vi "TS Acq Start.vi"(8 "error in":errorcluster, 11 "Water Tunnel Test Stand in":refnum<class "Water Tunnel Test Stand.lvclass">) -> (0 "error out":errorcluster, 3 "Water Tunnel Test Stand out":refnum<class "Water Tunnel Test Stand.lvclass">)   [LabVIEW 2019, in "Test Stands.lvlib" / "Water Tunnel Test Stand.lvclass"]
uses:
  Water Tunnel Test Stand.lvclass
  Results/Results Method.ctl
  Results/Results.lvlib
  Results/Water Tunnel Results/Water Tunnel Results.lvclass
  Generic Test Stand/TS Panel Method.ctl
  Generic Test Stand/Generic Test Stand.lvclass
  DAC/Water Tunnel/Traverse/DAC Traverse.lvclass
  C:/Users/wg/Documents/LV_Projects/test-stand/App/DAC/DAC.lvclass
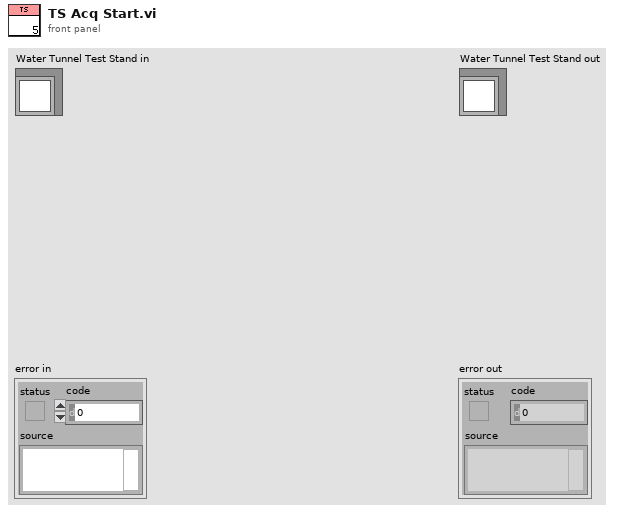
[diagram p1: front panel]
types:
  T1 = typedef "Generic Test Stand.lvclass/TS Panel Method.ctl" = enum16{"Send to Panel", "Receive from Panel"}
  T2 = typedef "Results.lvlib/Results Method.ctl" = enum16{"Get", "Set"}
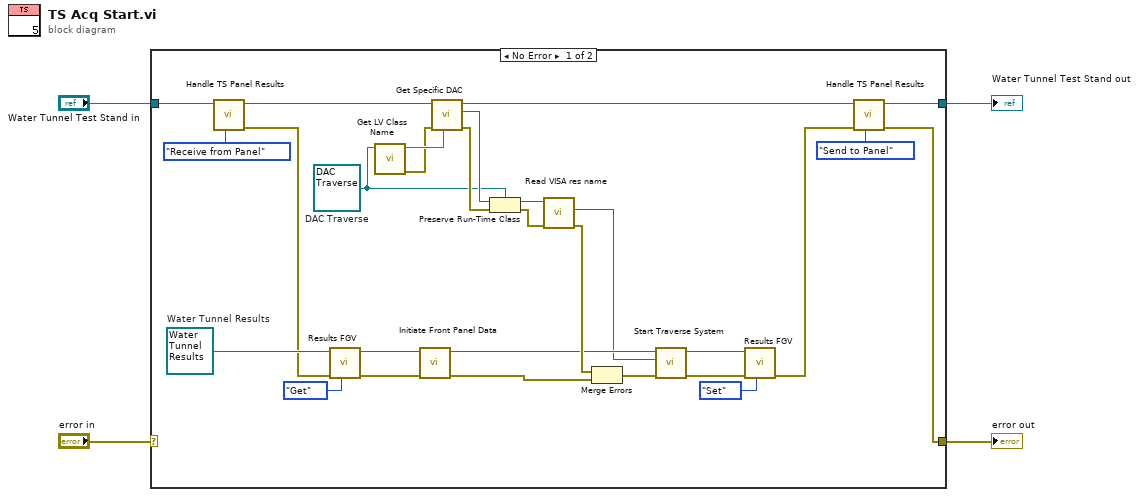
[diagram p0: block diagram]
diagram:
  n1 = case shown="No Error" "error in" {
    selector: "error in" -> [_ w34]
    tunnel: [w21 w34] -> w2
    tunnel: [w24 w33] -> w3
    tunnel: "Water Tunnel Test Stand in" -> [w25 w33]
    frame No Error {
      w15 = refnum<class "DAC Traverse.lvclass"> refnum  # DAC Traverse
      w30 = refnum<class "Water Tunnel Results.lvclass"> refnum  # Water Tunnel Results
      n2 = call-dynamic "Handle TS Panel Results.vi"("Method"=TS_Panel_Method."Receive from Panel", "Water Tunnel Test Stand in"=w25) -> ("error out"=w23:errorcluster, "Water Tunnel Test Stand out"=w20:refnum<class "Water Tunnel Test Stand.lvclass">)  [unwired: 8 in]
      n3 = call-dynamic "Results FGV.vi"("Method"=Results_Method."Get", "error in"=w23, "Water Tunnel Results in"=w30) -> ("error out"=w28:errorcluster, "Water Tunnel  Results out"=w29:refnum<class "Water Tunnel Results.lvclass">)  [unwired: 7 in]
      n4 = call <vilib>:"Get LV Class Name.vi"("object"=w15) -> ("error out"=w18:errorcluster, "class name"=w19:string)  [unwired: 9 in]
      n5 = call "Initiate Front Panel Data.vi"("error in"=w28, "Water Tunnel Results in"=w29) -> ("error out"=w11:errorcluster, "Water Tunnel Results out"=w7:refnum<class "Water Tunnel Results.lvclass">)  [unwired: 8 in]
      n6 = call-dynamic "Get Specific DAC.vi"("DAC Class Name"=w19, "error in"=w18, "Generic Test Stand in"=w20) -> ("error out"=w16:errorcluster, "DAC"=w17:refnum<class "DAC.lvclass">, "Generic Test Stand out"=w12:refnum<class "Water Tunnel Test Stand.lvclass">)  [unwired: 6 in]
      n7 = Preserve Run-Time Class(object in=w17, error in=w16, 2:w15) -> (object out=w14:refnum<class "DAC Traverse.lvclass">, error out=w13:errorcluster)
      n8 = call "Read VISA res name.vi"("error in (no error)"=w13, "DAC Traverse in"=w14) -> ("error out"=w10:errorcluster, "VISA res name"=w6:refnum<visa-resource-name>)  [unwired: 7 in, 1 out]
      n9 = Merge Errors(w10, w11) -> (w9:errorcluster)
      n10 = call "Start Traverse System.vi"("error in"=w9, "VISA resource name"=w6, "Water Tunnel Results in"=w7) -> ("error out"=w8:errorcluster, "Water Tunnel Results out"=w5:refnum<class "Water Tunnel Results.lvclass">)  [unwired: 7 in]
      n11 = call-dynamic "Results FGV.vi"("Method"=Results_Method."Set", "error in"=w8, "Water Tunnel Results in"=w5) -> ("error out"=w22:errorcluster)  [unwired: 7 in, 1 out]
      n12 = call-dynamic "Handle TS Panel Results.vi"("Method"=TS_Panel_Method."Send to Panel", "error in"=w22, "Water Tunnel Test Stand in"=w12) -> ("error out"=w21:errorcluster, "Water Tunnel Test Stand out"=w24:refnum<class "Water Tunnel Test Stand.lvclass">)  [unwired: 7 in]
    }
    frame Error {
    }
  }
  "error out" <- w2
  "Water Tunnel Test Stand out" <- w3
